vi "CAN Frames Read.vi"(7 "Channel Number":u32, 8 "error in (no error)":errorcluster, 9 "timeout [ms]":u32=100, 11 "FPGA Refnum":T1) -> (0 "error out":errorcluster, 1 "Valid":bool, 2 "Frames":T2[](array[typedef]) {"payload" format="%x"; "timestamp" format="%<%.7X\n%x>T"; "type" items=["CAN Data"=0, "CAN Remote"=1, "CAN Bus Error"=2, "CAN 2.0 Data"=8, "CAN FD Data"=16, "CAN FD+BRS Data"=24, "J1939 Data"=192, "Delay"=224, "Log Trigger"=225, "Start Trigger"=226]; "identifier" format="%x"})   [LabVIEW 2020, in "985x Support Addon Engine.lvlib"]
uses:
  985x Support Addon Engine.lvlib
  <vilib>/xnet/xnet.llb/XNET Frame CAN.ctl
  <vilib>/xnet/xnet.llb/XNET Frame Type CAN.ctl
  Types/FPGA Refnum.ctl
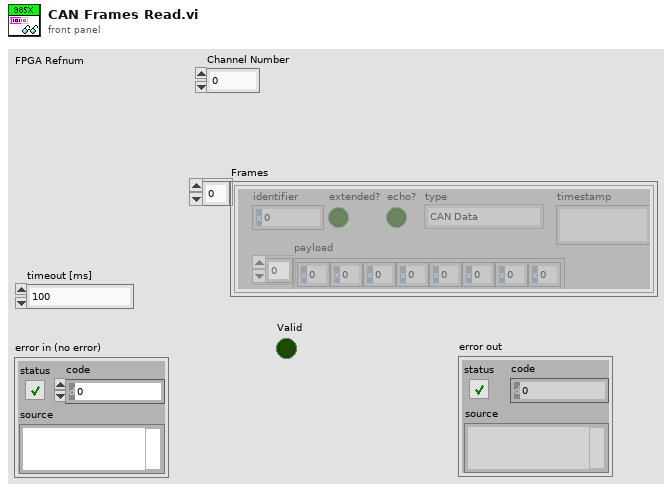
[diagram p1: front panel]
types:
  T1 = typedef "985x Support Addon Engine.lvlib/FPGA Refnum.ctl" = refnum<k20>
  T2 = typedef "XNET Frame CAN.ctl" = cluster{"timestamp":timestamp, "payload":u8[], "identifier":u32, "type":T3, "extended?":bool, "echo?":bool}
  T3 = typedef "XNET Frame Type CAN.ctl" = u8
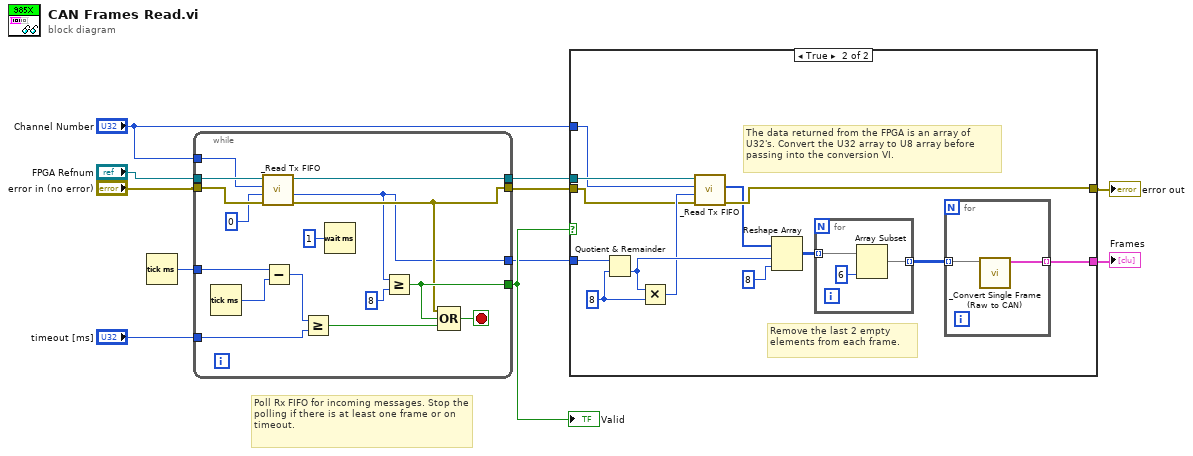
[diagram p0: block diagram]
diagram:
  # "Poll Rx FIFO for incoming messages. Stop the polling if there is at least one frame or on timeout."
  n1 = Tick Count (ms)() -> (millisecond timer value=w11:u32)
  n2 = while {
    tunnel: "FPGA Refnum" -> [w27]
    tunnel: "error in (no error)" -> [w26]
    tunnel: w11 -> [w24]
    tunnel: "timeout [ms]" -> [w21]
    tunnel: [w19] -> w9
    tunnel: [w16] -> w7
    tunnel: [w15] -> w8
    tunnel: [w12] -> w6
    tunnel: "Channel Number" -> [w14]
    stop <- w17 stop-if-true
    n3 = Tick Count (ms)() -> (millisecond timer value=w23:u32)
    n4 = call "_Read Tx FIFO.vi"("error in (no error)"=w26, "Number of elements"=u32 0, "Channel Number"=w14, "Refnum in"=w27) -> ("error out"=w15:errorcluster, "Elements Remaining"=w12:u32, "Refnum out"=w16:T1)  [unwired: 4 in, 1 out]
    n5 = Subtract(x=w24, y=w23) -> (x-y=w22:u32)
    n6 = Greater Or Equal?(x=w22, y=w21) -> (x >= y?=w18:bool)
    n7 = Wait (ms)(milliseconds to wait=u32 1) -> ()  [unwired: 1 out]
    n8 = Greater Or Equal?(x=w12, y=u32 8) -> (x >= y?=w19:bool)
    n9 = Compound Arithmetic op=OR(w15, w19, w18) -> (w17:bool)
  }
  "Valid" <- w9
  n10 = case shown="True" w9 {
    tunnel: [w28 w30] -> w5
    tunnel: w8 -> [w28 w31]
    tunnel: w7 -> [_ w34]
    tunnel: w6 -> [_ w41]
    tunnel: [_ w35] -> w4
    tunnel: "Channel Number" -> [_ w33]
    frame False {
    }
    frame True {
      w40 = u32 8 ("y")
      # "The data returned from the FPGA is an array of U32's. Convert the U32 array to U8 array before passing into the conversion VI."
      # "Remove the last 2 empty elements from each frame."
      n11 = Quotient & Remainder(x=w41, y=w40) -> (floor(x/y)=w37:u32)  [unwired: 1 out]
      n12 = Multiply(x=w37, y=w40) -> (x*y=w32:u32)
      n13 = call "_Read Tx FIFO.vi"("error in (no error)"=w31, "Number of elements"=w32, "Channel Number"=w33, "Refnum in"=w34) -> ("error out"=w30:errorcluster, "Data"=w29:u32[])  [unwired: 4 in, 2 out]
      n14 = Reshape Array(w29, w37, 8 ("y")) -> (w38:u32[][])
      n15 = for {
        tunnel: w38 -> [w46] mode=indexing
        tunnel: [w44] -> w36 mode=indexing
        n16 = Array Subset(array=w46, length=6) -> (w44:u32[])  [unwired: 1 in]
      }
      n17 = for {
        tunnel: w36 -> [w42] mode=indexing
        tunnel: [w43] -> w35 mode=indexing
        n18 = call "_Convert Single Frame (Raw to CAN).vi"("Raw U32"=w42) -> ("CAN frame"=w43:T2)  [unwired: 8 in, 1 out]
      }
    }
  }
  "error out" <- w5
  "Frames" <- w4
